vi "FuncVI_Sub - VI - Convert CE data to LV data (FlatStr to FlatStr).vi"(5 "CE data type":T1=enum."Unknown data type", 6 "error in":errorcluster, 8 "LV Type Descriptor":i16[](array[numeric]) format="%.0x", 9 "flattened data in":string) -> (0 "error out":errorcluster, 3 "flattened data out":string)   [LabVIEW 2021]
doc: "::: CalcExpress Toolkit :::\nCopyright (c) 2000-2026 Konstantin Shifershteyn. All rights reserved."
uses:
  cetypes.llb/CalcExpress Data Type.ctl
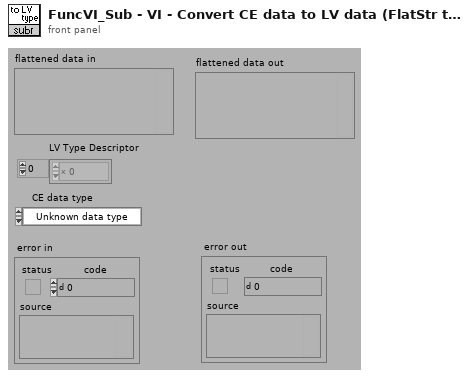
[diagram p1: front panel]
types:
  T1 = typedef "CalcExpress Data Type.ctl" = enum32{"String", "DBL Number", "identifier", "1D Array of DBL", "2D Array of DBL", "CDB Number", "1D Array of CDB", "2D Array of CDB", "1D Array of String", "2D Array of String", "Unknown data type"}
  T2 = enum16{"???", "int8", "int16", "int32", "float32", "float64", "float128", "complex32", "complex64", "complex128", "bool", "string", "path"}
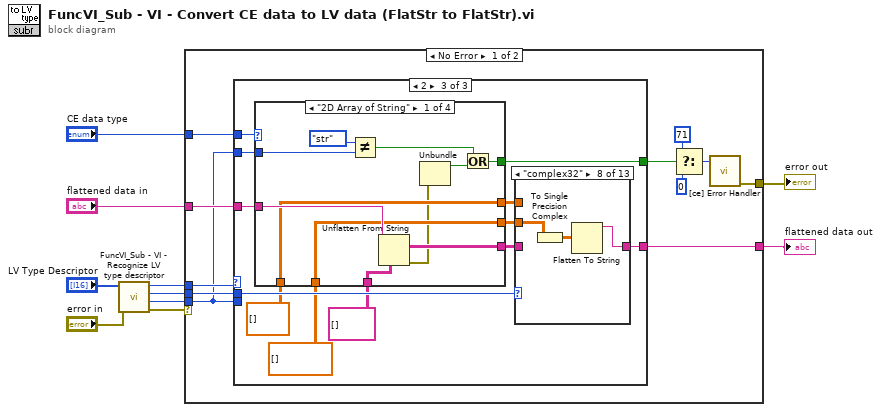
[diagram p0: block diagram]
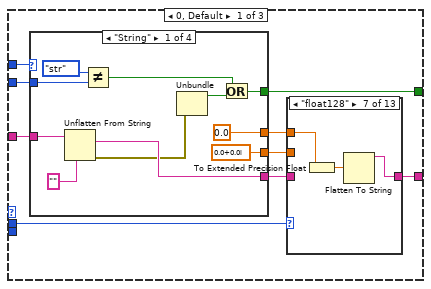
[diagram p2: hidden frame]
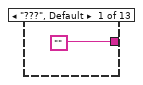
[diagram p3: hidden frame]
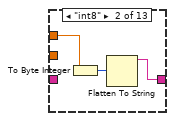
[diagram p4: hidden frame]
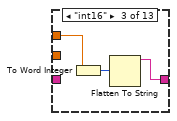
[diagram p5: hidden frame]
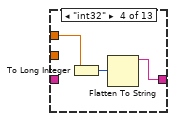
[diagram p6: hidden frame]
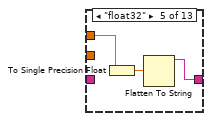
[diagram p7: hidden frame]
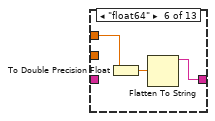
[diagram p8: hidden frame]
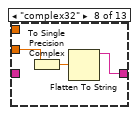
[diagram p9: hidden frame]
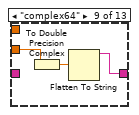
[diagram p10: hidden frame]
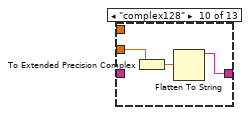
[diagram p11: hidden frame]
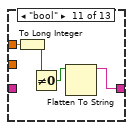
[diagram p12: hidden frame]
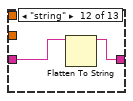
[diagram p13: hidden frame]
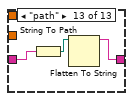
[diagram p14: hidden frame]
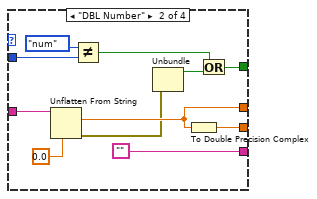
[diagram p15: hidden frame]
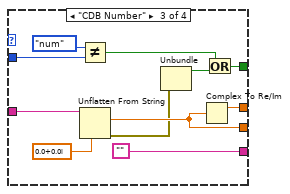
[diagram p16: hidden frame]
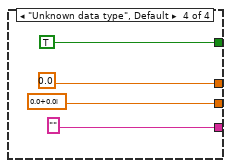
[diagram p17: hidden frame]
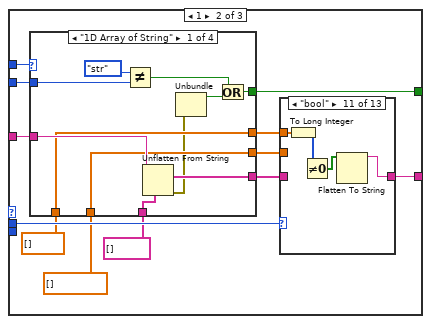
[diagram p18: hidden frame]
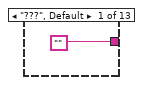
[diagram p19: hidden frame]
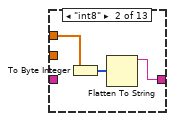
[diagram p20: hidden frame]
diagram:
  n1 = call "FuncVI_Sub - VI - Recognize LV type descriptor.vi"("error in"="error in", "Type Descriptor"="LV Type Descriptor") -> ("error out"=w1:errorcluster, "category"=w4:enum16{"num", "str"}, "representation"=w8:T2, "nDims"=w6:i32)  [unwired: 4 in]
  n2 = case shown="No Error" w1 {
    selector: w1 -> [_ w277]
    tunnel: w8 -> [w21 _]
    tunnel: "flattened data in" -> [w20 w278]
    tunnel: w6 -> [w19 _]
    tunnel: "CE data type" -> [w18 _]
    tunnel: w4 -> [w14 _]
    tunnel: [w17 w278] -> w3
    tunnel: [w11 w277] -> w2
    frame No Error {
      n3 = case shown="2" w19 {
        tunnel: w21 -> [w27 w113 w199]
        tunnel: w20 -> [w29 w115 w201]
        tunnel: w18 -> [w30 w116 w202]
        tunnel: w14 -> [_ _ _]
        tunnel: [w26 w112 w198] -> w17
        tunnel: [w28 w114 w200] -> w13
        tunnel: w14 -> [w24 w110 w196]
        frame 0, Default {
          n4 = case shown="\"String\"" w30 {
            tunnel: w29 -> [w78 w89 w100 _]
            tunnel: [w76 "" "" ""] -> w22
            tunnel: [0.0 w87 w97 0.0] -> w25
            tunnel: [cdb 0.0+0.0i w86 w96 cdb 0.0+0.0i] -> w23
            tunnel: [w69 w82 w91 TRUE ("err")] -> w28
            tunnel: w24 -> [w73 w81 w93 _]
            frame "String" {
              n5 = Unflatten From String(type="", binary string=w78) -> (value=w76:string, error out=w68:errorcluster)  [unwired: 3 in, 1 out]
              n6 = Not Equal?(x=enum16{"num", "str"}."str" ("y"), y=w73) -> (x != y?=w70:bool)
              n7 = Unbundle(w68) -> ("status"=w71:bool)  [unwired: 2 out]
              n8 = Or(x=w70, y=w71) -> (x .or. y?=w69:bool)
            }
            frame "DBL Number" {
              n9 = Unflatten From String(type=0.0, binary string=w89) -> (value=w87:dbl, error out=w79:errorcluster)  [unwired: 3 in, 1 out]
              n10 = Not Equal?(x=enum16{"num", "str"}."num" ("y"), y=w81) -> (x != y?=w83:bool)
              n11 = Unbundle(w79) -> ("status"=w80:bool)  [unwired: 2 out]
              n12 = To Double Precision Complex(1:w87) -> (0:w86:cdb)
              n13 = Or(x=w83, y=w80) -> (x .or. y?=w82:bool)
            }
            frame "CDB Number" {
              n14 = Not Equal?(x=enum16{"num", "str"}."num" ("y"), y=w93) -> (x != y?=w94:bool)
              n15 = Unflatten From String(type=cdb 0.0+0.0i, binary string=w100) -> (value=w96:cdb, error out=w90:errorcluster)  [unwired: 3 in, 1 out]
              n16 = Unbundle(w90) -> ("status"=w92:bool)  [unwired: 2 out]
              n17 = Complex To Re/Im(x + iy=w96) -> (x=w97:dbl)  [unwired: 1 out]
              n18 = Or(x=w94, y=w92) -> (x .or. y?=w91:bool)
            }
            frame "Unknown data type", Default {
            }
          }
          n19 = case shown="\"float128\"" w27 {
            tunnel: ["" w34 w37 w40 w43 w46 w49 w52 w55 w58 w62 w64 w67] -> w26
            tunnel: w25 -> [_ w33 w36 w39 w42 w45 w48 _ _ _ w61 _ _]
            tunnel: w23 -> [_ _ _ _ _ _ _ w50 w53 w56 _ _ _]
            tunnel: w22 -> [_ _ _ _ _ _ _ _ _ _ _ w63 w66]
            frame "???", Default {
            }
            frame "int8" {
              n20 = To Byte Integer(number=w33) -> (8bit integer=w32:i8)
              n21 = Flatten To String(anything=w32) -> (data string=w34:string)  [unwired: 3 in, 2 out]
            }
            frame "int16" {
              n22 = To Word Integer(number=w36) -> (16bit integer=w35:i16)
              n23 = Flatten To String(anything=w35) -> (data string=w37:string)  [unwired: 3 in, 2 out]
            }
            frame "int32" {
              n24 = To Long Integer(number=w39) -> (32bit integer=w38:i32)
              n25 = Flatten To String(anything=w38) -> (data string=w40:string)  [unwired: 3 in, 2 out]
            }
            frame "float32" {
              n26 = To Single Precision Float(number=w42) -> (single precision float=w41:sgl)
              n27 = Flatten To String(anything=w41) -> (data string=w43:string)  [unwired: 3 in, 2 out]
            }
            frame "float64" {
              n28 = To Double Precision Float(number=w45) -> (double precision float=w44:dbl)
              n29 = Flatten To String(anything=w44) -> (data string=w46:string)  [unwired: 3 in, 2 out]
            }
            frame "float128" {
              n30 = To Extended Precision Float(1:w48) -> (0:w47:ext)
              n31 = Flatten To String(anything=w47) -> (data string=w49:string)  [unwired: 3 in, 2 out]
            }
            frame "complex32" {
              n32 = To Single Precision Complex(1:w50) -> (0:w51:csg)
              n33 = Flatten To String(anything=w51) -> (data string=w52:string)  [unwired: 3 in, 2 out]
            }
            frame "complex64" {
              n34 = To Double Precision Complex(1:w53) -> (0:w54:cdb)
              n35 = Flatten To String(anything=w54) -> (data string=w55:string)  [unwired: 3 in, 2 out]
            }
            frame "complex128" {
              n36 = To Extended Precision Complex(1:w56) -> (0:w57:cxt)
              n37 = Flatten To String(anything=w57) -> (data string=w58:string)  [unwired: 3 in, 2 out]
            }
            frame "bool" {
              n38 = To Long Integer(number=w61) -> (32bit integer=w60:i32)
              n39 = Not Equal To 0?(x=w60) -> (x != 0?=w59:bool)
              n40 = Flatten To String(anything=w59) -> (data string=w62:string)  [unwired: 3 in, 2 out]
            }
            frame "string" {
              n41 = Flatten To String(anything=w63) -> (data string=w64:string)  [unwired: 3 in, 2 out]
            }
            frame "path" {
              n42 = String To Path(string=w66) -> (path=w65:path)
              n43 = Flatten To String(anything=w65) -> (data string=w67:string)  [unwired: 3 in, 2 out]
            }
          }
        }
        frame 1 {
          n44 = case shown="\"1D Array of String\"" w116 {
            tunnel: w115 -> [w164 w175 w186 _]
            tunnel: [w163 w166 w177 w189] -> w108
            tunnel: [w155 w174 w185 w187] -> w111
            tunnel: [w156 w173 w184 w188] -> w109
            tunnel: [w158 w170 w179 TRUE ("err")] -> w114
            tunnel: w110 -> [w162 w169 w181 _]
            tunnel: string[] [] -> [w157 w166 w177 w189]
            tunnel: cdb[] [] -> [w156 _ w178 w188]
            tunnel: dbl[] [] -> [w155 w167 _ w187]
            frame "1D Array of String" {
              n45 = Not Equal?(x=enum16{"num", "str"}."str" ("y"), y=w162) -> (x != y?=w159:bool)
              n46 = Unflatten From String(type=w157, binary string=w164) -> (value=w163:string[], error out=w154:errorcluster)  [unwired: 3 in, 1 out]
              n47 = Unbundle(w154) -> ("status"=w160:bool)  [unwired: 2 out]
              n48 = Or(x=w159, y=w160) -> (x .or. y?=w158:bool)
            }
            frame "1D Array of DBL" {
              n49 = Unflatten From String(type=w167, binary string=w175) -> (value=w174:dbl[], error out=w165:errorcluster)  [unwired: 3 in, 1 out]
              n50 = Not Equal?(x=enum16{"num", "str"}."num" ("y"), y=w169) -> (x != y?=w171:bool)
              n51 = Unbundle(w165) -> ("status"=w168:bool)  [unwired: 2 out]
              n52 = To Double Precision Complex(1:w174) -> (0:w173:cdb[])
              n53 = Or(x=w171, y=w168) -> (x .or. y?=w170:bool)
            }
            frame "1D Array of CDB" {
              n54 = Unflatten From String(type=w178, binary string=w186) -> (value=w184:cdb[], error out=w176:errorcluster)  [unwired: 3 in, 1 out]
              n55 = Not Equal?(x=enum16{"num", "str"}."num" ("y"), y=w181) -> (x != y?=w182:bool)
              n56 = Unbundle(w176) -> ("status"=w180:bool)  [unwired: 2 out]
              n57 = Complex To Re/Im(x + iy=w184) -> (x=w185:dbl[])  [unwired: 1 out]
              n58 = Or(x=w182, y=w180) -> (x .or. y?=w179:bool)
            }
            frame "Unknown data type", Default {
            }
          }
          n59 = case shown="\"bool\"" w113 {
            tunnel: ["" w120 w123 w126 w129 w132 w135 w138 w141 w144 w148 w150 w153] -> w112
            tunnel: w111 -> [_ w119 w122 w125 w128 w131 w134 _ _ _ w147 _ _]
            tunnel: w109 -> [_ _ _ _ _ _ _ w136 w139 w142 _ _ _]
            tunnel: w108 -> [_ _ _ _ _ _ _ _ _ _ _ w149 w152]
            frame "???", Default {
            }
            frame "int8" {
              n60 = To Byte Integer(number=w119) -> (8bit integer=w118:i8[])
              n61 = Flatten To String(anything=w118) -> (data string=w120:string)  [unwired: 3 in, 2 out]
            }
            frame "int16" {
              n62 = To Word Integer(number=w122) -> (16bit integer=w121:i16[])
              n63 = Flatten To String(anything=w121) -> (data string=w123:string)  [unwired: 3 in, 2 out]
            }
            frame "int32" {
              n64 = To Long Integer(number=w125) -> (32bit integer=w124:i32[])
              n65 = Flatten To String(anything=w124) -> (data string=w126:string)  [unwired: 3 in, 2 out]
            }
            frame "float32" {
              n66 = To Single Precision Float(number=w128) -> (single precision float=w127:sgl[])
              n67 = Flatten To String(anything=w127) -> (data string=w129:string)  [unwired: 3 in, 2 out]
            }
            frame "float64" {
              n68 = To Double Precision Float(number=w131) -> (double precision float=w130:dbl[])
              n69 = Flatten To String(anything=w130) -> (data string=w132:string)  [unwired: 3 in, 2 out]
            }
            frame "float128" {
              n70 = To Extended Precision Float(1:w134) -> (0:w133:ext[])
              n71 = Flatten To String(anything=w133) -> (data string=w135:string)  [unwired: 3 in, 2 out]
            }
            frame "complex32" {
              n72 = To Single Precision Complex(1:w136) -> (0:w137:csg[])
              n73 = Flatten To String(anything=w137) -> (data string=w138:string)  [unwired: 3 in, 2 out]
            }
            frame "complex64" {
              n74 = To Double Precision Complex(1:w139) -> (0:w140:cdb[])
              n75 = Flatten To String(anything=w140) -> (data string=w141:string)  [unwired: 3 in, 2 out]
            }
            frame "complex128" {
              n76 = To Extended Precision Complex(1:w142) -> (0:w143:cxt[])
              n77 = Flatten To String(anything=w143) -> (data string=w144:string)  [unwired: 3 in, 2 out]
            }
            frame "bool" {
              n78 = To Long Integer(number=w147) -> (32bit integer=w146:i32[])
              n79 = Not Equal To 0?(x=w146) -> (x != 0?=w145:bool[])
              n80 = Flatten To String(anything=w145) -> (data string=w148:string)  [unwired: 3 in, 2 out]
            }
            frame "string" {
              n81 = Flatten To String(anything=w149) -> (data string=w150:string)  [unwired: 3 in, 2 out]
            }
            frame "path" {
              n82 = String To Path(string=w152) -> (path=w151:path[])
              n83 = Flatten To String(anything=w151) -> (data string=w153:string)  [unwired: 3 in, 2 out]
            }
          }
        }
        frame 2 {
          n84 = case shown="\"2D Array of String\"" w202 {
            tunnel: w201 -> [w250 w261 w272 _]
            tunnel: [w249 w252 w263 w275] -> w194
            tunnel: [w241 w260 w271 w273] -> w197
            tunnel: [w242 w259 w270 w274] -> w195
            tunnel: [w244 w256 w265 TRUE ("err")] -> w200
            tunnel: w196 -> [w248 w255 w267 _]
            tunnel: string[][] [] -> [w243 w252 w263 w275]
            tunnel: cdb[][] [] -> [w242 _ w264 w274]
            tunnel: dbl[][] [] -> [w241 w253 _ w273]
            frame "2D Array of String" {
              n85 = Not Equal?(x=enum16{"num", "str"}."str" ("y"), y=w248) -> (x != y?=w245:bool)
              n86 = Unflatten From String(type=w243, binary string=w250) -> (value=w249:string[][], error out=w240:errorcluster)  [unwired: 3 in, 1 out]
              n87 = Unbundle(w240) -> ("status"=w246:bool)  [unwired: 2 out]
              n88 = Or(x=w245, y=w246) -> (x .or. y?=w244:bool)
            }
            frame "2D Array of DBL" {
              n89 = Not Equal?(x=enum16{"num", "str"}."num" ("y"), y=w255) -> (x != y?=w257:bool)
              n90 = Unflatten From String(type=w253, binary string=w261) -> (value=w260:dbl[][], error out=w251:errorcluster)  [unwired: 3 in, 1 out]
              n91 = Unbundle(w251) -> ("status"=w254:bool)  [unwired: 2 out]
              n92 = To Double Precision Complex(1:w260) -> (0:w259:cdb[][])
              n93 = Or(x=w257, y=w254) -> (x .or. y?=w256:bool)
            }
            frame "2D Array of CDB" {
              n94 = Not Equal?(x=enum16{"num", "str"}."num" ("y"), y=w267) -> (x != y?=w268:bool)
              n95 = Unflatten From String(type=w264, binary string=w272) -> (value=w270:cdb[][], error out=w262:errorcluster)  [unwired: 3 in, 1 out]
              n96 = Unbundle(w262) -> ("status"=w266:bool)  [unwired: 2 out]
              n97 = Or(x=w268, y=w266) -> (x .or. y?=w265:bool)
              n98 = Complex To Re/Im(x + iy=w270) -> (x=w271:dbl[][])  [unwired: 1 out]
            }
            frame "Unknown data type", Default {
            }
          }
          n99 = case shown="\"complex32\"" w199 {
            tunnel: ["" w206 w209 w212 w215 w218 w221 w224 w227 w230 w234 w236 w239] -> w198
            tunnel: w197 -> [_ w205 w208 w211 w214 w217 w220 _ _ _ w233 _ _]
            tunnel: w195 -> [_ _ _ _ _ _ _ w222 w225 w228 _ _ _]
            tunnel: w194 -> [_ _ _ _ _ _ _ _ _ _ _ w235 w238]
            frame "???", Default {
            }
            frame "int8" {
              n100 = To Byte Integer(number=w205) -> (8bit integer=w204:i8[][])
              n101 = Flatten To String(anything=w204) -> (data string=w206:string)  [unwired: 3 in, 2 out]
            }
            frame "int16" {
              n102 = To Word Integer(number=w208) -> (16bit integer=w207:i16[][])
              n103 = Flatten To String(anything=w207) -> (data string=w209:string)  [unwired: 3 in, 2 out]
            }
            frame "int32" {
              n104 = To Long Integer(number=w211) -> (32bit integer=w210:i32[][])
              n105 = Flatten To String(anything=w210) -> (data string=w212:string)  [unwired: 3 in, 2 out]
            }
            frame "float32" {
              n106 = To Single Precision Float(number=w214) -> (single precision float=w213:sgl[][])
              n107 = Flatten To String(anything=w213) -> (data string=w215:string)  [unwired: 3 in, 2 out]
            }
            frame "float64" {
              n108 = To Double Precision Float(number=w217) -> (double precision float=w216:dbl[][])
              n109 = Flatten To String(anything=w216) -> (data string=w218:string)  [unwired: 3 in, 2 out]
            }
            frame "float128" {
              n110 = To Extended Precision Float(1:w220) -> (0:w219:ext[][])
              n111 = Flatten To String(anything=w219) -> (data string=w221:string)  [unwired: 3 in, 2 out]
            }
            frame "complex32" {
              n112 = To Single Precision Complex(1:w222) -> (0:w223:csg[][])
              n113 = Flatten To String(anything=w223) -> (data string=w224:string)  [unwired: 3 in, 2 out]
            }
            frame "complex64" {
              n114 = To Double Precision Complex(1:w225) -> (0:w226:cdb[][])
              n115 = Flatten To String(anything=w226) -> (data string=w227:string)  [unwired: 3 in, 2 out]
            }
            frame "complex128" {
              n116 = To Extended Precision Complex(1:w228) -> (0:w229:cxt[][])
              n117 = Flatten To String(anything=w229) -> (data string=w230:string)  [unwired: 3 in, 2 out]
            }
            frame "bool" {
              n118 = To Long Integer(number=w233) -> (32bit integer=w232:i32[][])
              n119 = Not Equal To 0?(x=w232) -> (x != 0?=w231:bool[][])
              n120 = Flatten To String(anything=w231) -> (data string=w234:string)  [unwired: 3 in, 2 out]
            }
            frame "string" {
              n121 = Flatten To String(anything=w235) -> (data string=w236:string)  [unwired: 3 in, 2 out]
            }
            frame "path" {
              n122 = String To Path(string=w238) -> (path=w237:path[][])
              n123 = Flatten To String(anything=w237) -> (data string=w239:string)  [unwired: 3 in, 2 out]
            }
          }
        }
      }
      n124 = Select(t=71, s=w13, f=0) -> (s? t:f=w12:i32)
      n125 = call "[ce] Error Handler.vi"("error code"=w12) -> ("error out"=w11:errorcluster)  [unwired: 9 in, 1 out]
    }
    frame Error {
    }
  }
  "flattened data out" <- w3
  "error out" <- w2
